vi "Ring_Styles_18.vi"() -> ()   [LabVIEW 2018]
doc: "Use this template to build a VI to use as a subVI."
uses:
  <vilib>/Utility/miscctls.llb/LVStringsAndValuesArrayTypeDef.ctl
panel:
  out "Strings And Values []":T1
  out "error out":errorcluster
  out "reference out":refnum<vi>
  in  "error in (no error)":errorcluster
  in  "reference":refnum<vi>
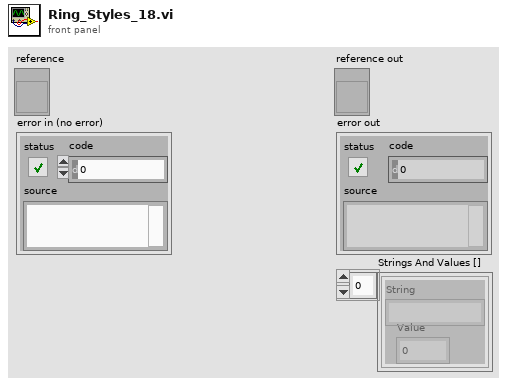
[diagram p1: front panel]
types:
  T1 = typedef "LVStringsAndValuesArrayTypeDef.ctl" = cluster{"String":string, "Value":ext}[]
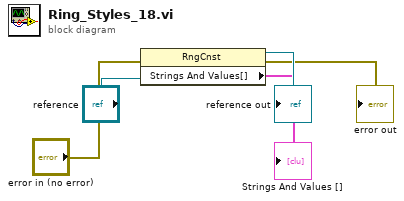
[diagram p0: block diagram]
diagram:
  n1 = property class="RngCnst"(reference="reference", error in="error in (no error)") -> (reference out=→"reference out":refnum<vi>, error out=→"error out":errorcluster, "Strings And Values[]"=→"Strings And Values []":T1)
